vi "GlobalValue.vi"() -> ()   [LabVIEW 2019]
panel:
  in  "Robotics:testbed:physical-ai-db":T1
  in  "CobotData":cluster{"data2":dbl[]}
  in  "StringData":string
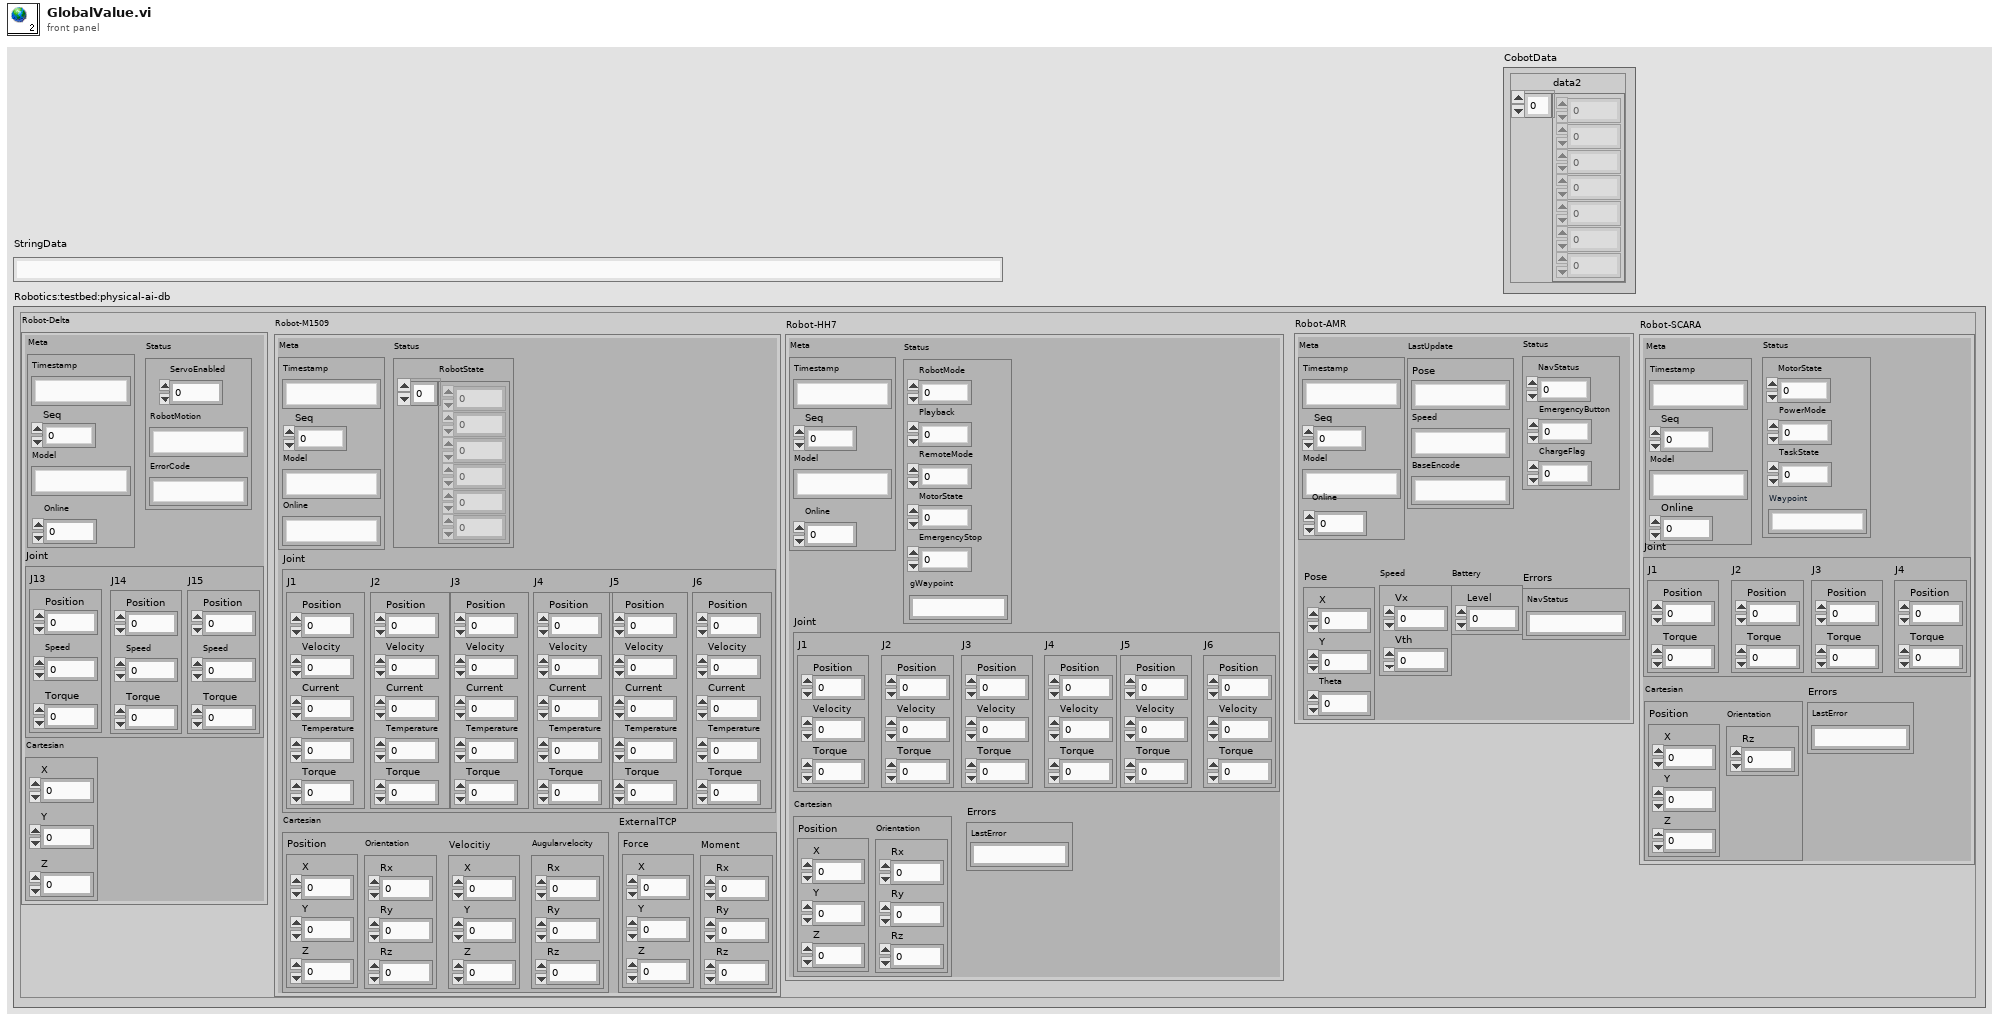
[diagram p1: front panel]
types:
  T1 = cluster{"Robot-Delta":cluster{"Meta":cluster{"Timestamp":string, "Seq":dbl, "Model":string, "Online":dbl}, "Status":cluster{"ServoEnabled":dbl, "RobotMotion":string, "ErrorCode":string}, "Joint":cluster{"J13":cluster{"Position":dbl, "Speed":dbl, "Torque":dbl}, "J14":cluster{"Position":dbl, "Speed":dbl, "Torque":dbl}, "J15":cluster{"Position":dbl, "Speed":dbl, "Torque":dbl}}, "Cartesian":cluster{"X":dbl, "Y":dbl, "Z":dbl}}, "Robot-M1509":cluster{"Meta":cluster{"Timestamp":string, "Seq":dbl, "Model":string, "Online":string}, "Status":cluster{"RobotState":dbl[]}, "Joint":cluster{"J1":cluster{"Position":dbl, "Velocity":dbl, "Current":dbl, "Temperature":dbl, "Torque":dbl}, "J2":cluster{"Position":dbl, "Velocity":dbl, "Current":dbl, "Temperature":dbl, "Torque":dbl}, "J3":cluster{"Position":dbl, "Velocity":dbl, "Current":dbl, "Temperature":dbl, "Torque":dbl}, "J4":cluster{"Position":dbl, "Velocity":dbl, "Current":dbl, "Temperature":dbl, "Torque":dbl}, "J5":cluster{"Position":dbl, "Velocity":dbl, "Current":dbl, "Temperature":dbl, "Torque":dbl}, "J6":cluster{"Position":dbl, "Velocity":dbl, "Current":dbl, "Temperature":dbl, "Torque":dbl}}, "Cartesian":cluster{"Position":cluster{"X":dbl, "Y":dbl, "Z":dbl}, "Orientation":cluster{"Rx":dbl, "Ry":dbl, "Rz":dbl}, "Velocitiy":cluster{"X":dbl, "Y":dbl, "Z":dbl}, "Augularvelocity":cluster{"Rx":dbl, "Ry":dbl, "Rz":dbl}}, "ExternalTCP":cluster{"Force":cluster{"X":dbl, "Y":dbl, "Z":dbl}, "Moment":cluster{"Rx":dbl, "Ry":dbl, "Rz":dbl}}}, "Robot-HH7":cluster{"Meta":cluster{"Timestamp":string, "Model":string, "Online":dbl, "Seq":dbl}, "Status":cluster{"RobotMode":dbl, "Playback":dbl, "RemoteMode":dbl, "MotorState":dbl, "EmergencyStop":dbl, "gWaypoint":string}, "Joint":cluster{"J1":cluster{"Position":dbl, "Velocity":dbl, "Torque":dbl}, "J2":cluster{"Position":dbl, "Velocity":dbl, "Torque":dbl}, "J3":cluster{"Position":dbl, "Velocity":dbl, "Torque":dbl}, "J4":cluster{"Position":dbl, "Velocity":dbl, "Torque":dbl}, "J5":cluster{"Position":dbl, "Velocity":dbl, "Torque":dbl}, "J6":cluster{"Position":dbl, "Velocity":dbl, "Torque":dbl}}, "Cartesian":cluster{"Position":cluster{"X":dbl, "Y":dbl, "Z":dbl}, "Orientation":cluster{"Rx":dbl, "Ry":dbl, "Rz":dbl}}, "Errors":cluster{"LastError":string}}, "Robot-AMR":cluster{"Meta":cluster{"Timestamp":string, "Seq":dbl, "Model":string, "Online":dbl}, "LastUpdate":cluster{"Pose":string, "Speed":string, "BaseEncode":string}, "Status":cluster{"NavStatus":dbl, "EmergencyButton":dbl, "ChargeFlag":dbl}, "Pose":cluster{"X":dbl, "Y":dbl, "Theta":dbl}, "Speed":cluster{"Vx":dbl, "Vth":dbl}, "Battery":cluster{"Level":dbl}, "Errors":cluster{"NavStatus":string}}, "Robot-SCARA":cluster{"Meta":cluster{"Timestamp":string, "Model":string, "Seq":dbl, "Online":dbl}, "Status":cluster{"MotorState":dbl, "PowerMode":dbl, "TaskState":dbl, "Waypoint":string}, "Joint":cluster{"J1":cluster{"Position":dbl, "Torque":dbl}, "J2":cluster{"Position":dbl, "Torque":dbl}, "J3":cluster{"Position":dbl, "Torque":dbl}, "J4":cluster{"Position":dbl, "Torque":dbl}}, "Cartesian":cluster{"Position":cluster{"X":dbl, "Y":dbl, "Z":dbl}, "Orientation":cluster{"Rz":dbl}}, "Errors":cluster{"LastError":string}}}
diagram:
